vi "serial.vi"() -> ()   [LabVIEW 2017]
uses:
  <vilib>/Instr/_visa.llb/VISA Configure Serial Port (Instr).vi
panel:
  out "SUICHE":bool
  out "TEMPERATURA":dbl(slide) scale=0.0..100.0
  out "read buffer":string
  in  "PARAR":bool
  in  "PUERTO":refnum<visa-resource-name>="COM4"
  in  "Izquierda":bool
  in  "Derecha":bool
  in  "VELOCIDAD":dbl(knob) scale=0.0..100.0
  in  "LED2":bool
  in  "LED1":bool
  in  "stop":bool
  # "GIRO"
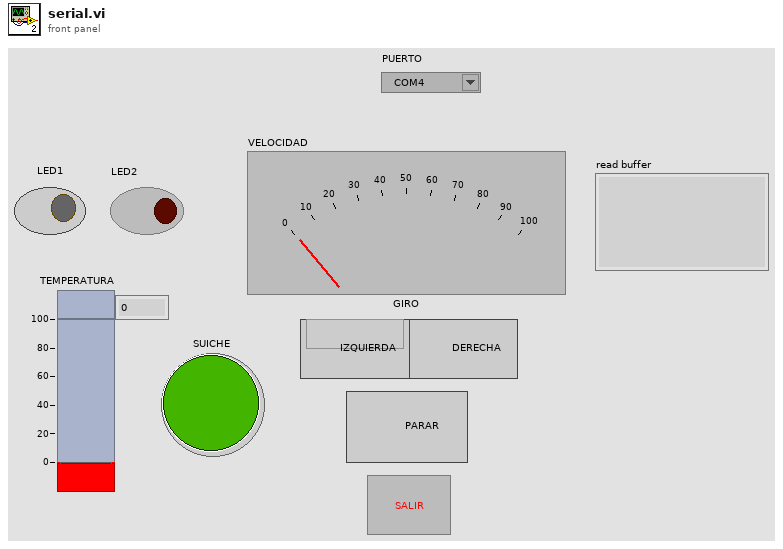
[diagram p1: front panel]
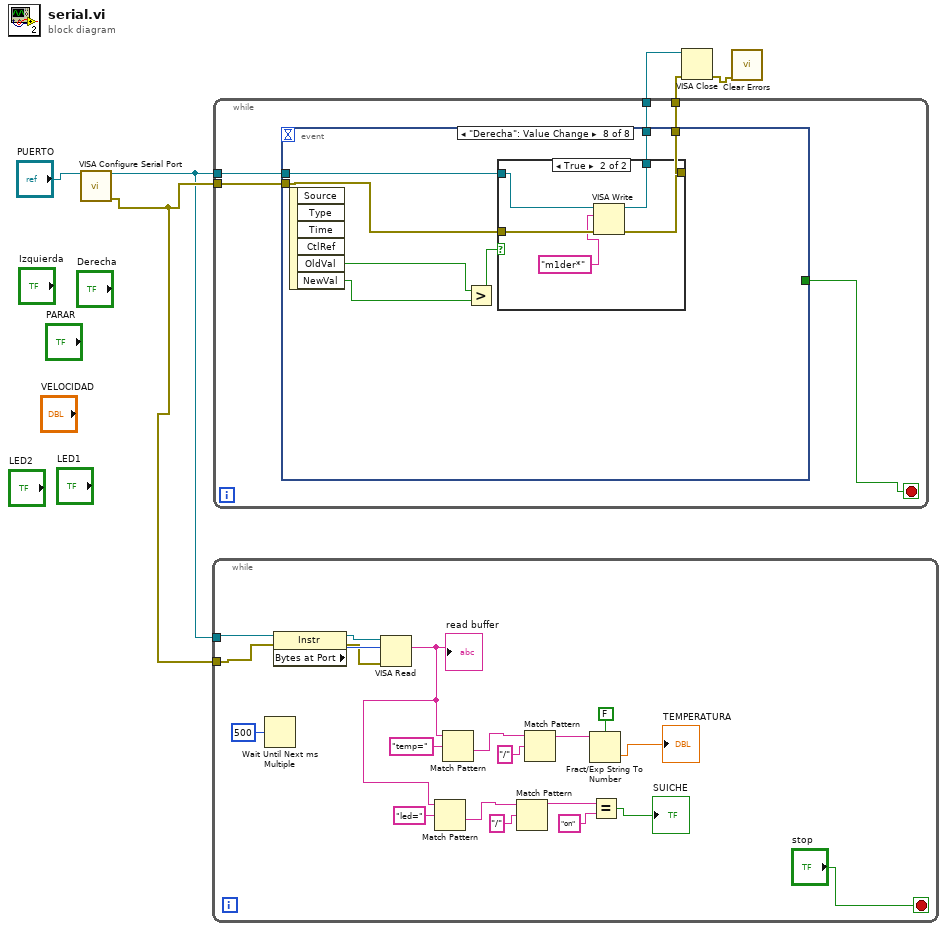
[diagram p0: block diagram]
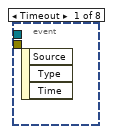
[diagram p2: hidden frame]
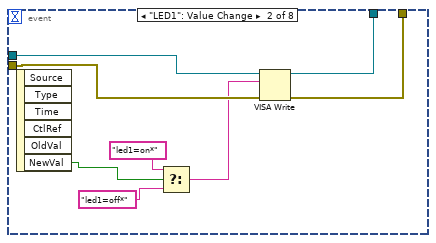
[diagram p3: hidden frame]
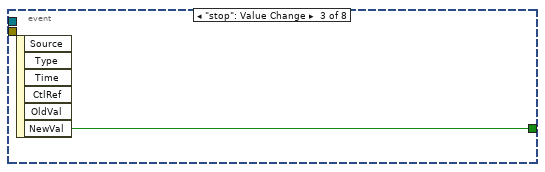
[diagram p4: hidden frame]
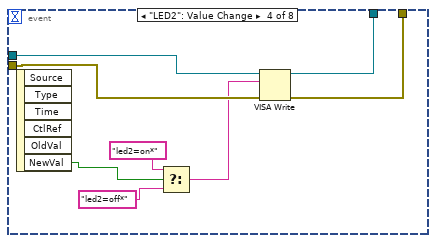
[diagram p5: hidden frame]
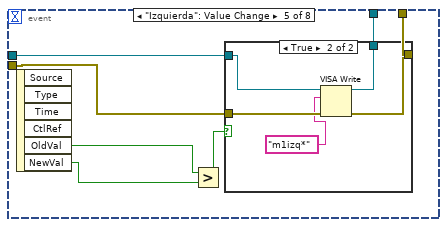
[diagram p6: hidden frame]
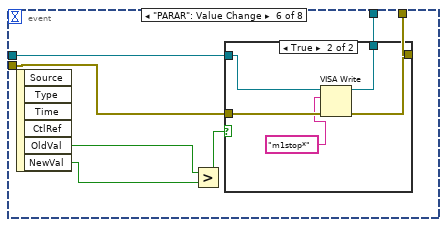
[diagram p8: hidden frame]
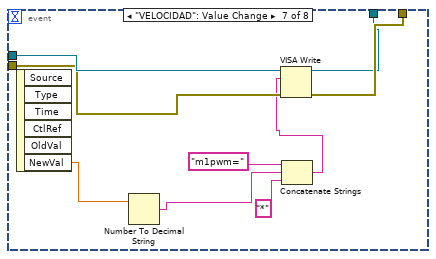
[diagram p10: hidden frame]
diagram:
  n1 = call-poly "VISA Configure Serial Port"("VISA resource name"="PUERTO") -> ("VISA resource name out"=w1:refnum<visa-resource-name>, "error out"=w2:errorcluster)  [unwired: 13 in]
  n2 = while {
    tunnel: w2 -> [w22]
    tunnel: w1 -> [w23]
    stop <- "stop" stop-if-true
    n3 = Wait Until Next ms Multiple(millisecond multiple=u32 500) -> ()  [unwired: 1 out]
    n4 = property class="Instr"(reference=w23, error in=w22) -> (reference out=w25:refnum<visa-resource-name>, error out=w24:errorcluster, "Bytes at Port"=w26:u32)
    n5 = VISA Read(VISA resource name=w25, byte count=w26, error in (no error)=w24) -> (read buffer=w9:string)  [unwired: 3 out]
    "read buffer" <- w9
    n6 = Match Pattern(string=w9, regular expression="led=") -> (after substring=w13:string)  [unwired: 1 in, 3 out]
    n7 = Match Pattern(string=w9, regular expression="temp=") -> (after substring=w19:string)  [unwired: 1 in, 3 out]
    n8 = Match Pattern(string=w13, regular expression="/") -> (before substring=w11:string)  [unwired: 1 in, 3 out]
    n9 = Match Pattern(string=w19, regular expression="/") -> (before substring=w17:string)  [unwired: 1 in, 3 out]
    n10 = Fract/Exp String To Number(use system decimal point (T)=FALSE, string=w17) -> (number=→"TEMPERATURA":dbl)  [unwired: 2 in, 1 out]
    n11 = Equal?(x=w11, y="on") -> (x = y?=→"SUICHE":bool)
  }
  n12 = while {
    tunnel: w1 -> [w31]
    tunnel: w2 -> [w30]
    tunnel: [w29] -> w5
    tunnel: [w28] -> w4
    stop <- w27 stop-if-true
    n13 = event shown="[7] \"Derecha\": Value Change" {
      selector: _ -> [_ _ _ _ _ _ _ _]
      dyn-events: _ -> [_ _ _ _ _ _ _ _]
      timeout: _ -> [_ _ _ _ _ _ _ _]
      tunnel: w31 -> [_ w39 _ w48 w55 w67 w81 w88]
      tunnel: w30 -> [_ w38 _ w47 w54 w66 w80 w87]
      tunnel: [_ w33 _ w42 w53 w65 w78 w86] -> w29
      tunnel: [_ w32 _ w41 w52 w64 w79 w85] -> w28
      tunnel: [_ _ w40 _ _ _ _ _] -> w27
      event Timeout {
        n14 = event-data() -> ()  [unwired: 1 in, 3 out]
      }
      event "LED1": Value Change {
        n15 = event-data() -> ("NewVal"=w37:bool)  [unwired: 1 in, 5 out]
        n16 = Select(t="led1=on*", s=w37, f="led1=off*") -> (s? t:f=w34:string)
        n17 = VISA Write(VISA resource name=w39, write buffer=w34, error in (no error)=w38) -> (VISA resource name out=w33:refnum<visa-resource-name>, error out=w32:errorcluster)  [unwired: 1 out]
      }
      event "stop": Value Change {
        n18 = event-data() -> ("NewVal"=w40:bool)  [unwired: 1 in, 5 out]
      }
      event "LED2": Value Change {
        n19 = event-data() -> ("NewVal"=w46:bool)  [unwired: 1 in, 5 out]
        n20 = Select(t="led2=on*", s=w46, f="led2=off*") -> (s? t:f=w43:string)
        n21 = VISA Write(VISA resource name=w48, write buffer=w43, error in (no error)=w47) -> (VISA resource name out=w42:refnum<visa-resource-name>, error out=w41:errorcluster)  [unwired: 1 out]
      }
      event "Izquierda": Value Change {
        n22 = event-data() -> ("OldVal"=w51:bool, "NewVal"=w50:bool)  [unwired: 1 in, 4 out]
        n23 = Greater?(x=w51, y=w50) -> (0:w49:bool)
        n24 = case shown="True" w49 {
          tunnel: w55 -> [_ w60]
          tunnel: w54 -> [_ w59]
          tunnel: [_ w58] -> w53
          tunnel: [_ w57] -> w52
          frame False {
          }
          frame True {
            n25 = VISA Write(VISA resource name=w60, write buffer="m1izq*", error in (no error)=w59) -> (VISA resource name out=w58:refnum<visa-resource-name>, error out=w57:errorcluster)  [unwired: 1 out]
          }
        }
      }
      event "PARAR": Value Change {
        n26 = event-data() -> ("OldVal"=w63:bool, "NewVal"=w62:bool)  [unwired: 1 in, 4 out]
        n27 = Greater?(x=w63, y=w62) -> (0:w61:bool)
        n28 = case shown="True" w61 {
          tunnel: w67 -> [_ w72]
          tunnel: w66 -> [_ w71]
          tunnel: [_ w70] -> w65
          tunnel: [_ w69] -> w64
          frame False {
          }
          frame True {
            n29 = VISA Write(VISA resource name=w72, write buffer="m1stop*", error in (no error)=w71) -> (VISA resource name out=w70:refnum<visa-resource-name>, error out=w69:errorcluster)  [unwired: 1 out]
          }
        }
      }
      event "VELOCIDAD": Value Change {
        n30 = event-data() -> ("NewVal"=w73:dbl)  [unwired: 1 in, 5 out]
        n31 = Number To Decimal String(number=w73) -> (decimal integer string=w76:string)  [unwired: 1 in]
        n32 = Concatenate Strings("m1pwm=" ("string"), w76, "*" ("string")) -> (w74:string)
        n33 = VISA Write(VISA resource name=w81, write buffer=w74, error in (no error)=w80) -> (VISA resource name out=w78:refnum<visa-resource-name>, error out=w79:errorcluster)  [unwired: 1 out]
      }
      event "Derecha": Value Change {
        n34 = event-data() -> ("OldVal"=w84:bool, "NewVal"=w83:bool)  [unwired: 1 in, 4 out]
        n35 = Greater?(x=w84, y=w83) -> (0:w82:bool)
        n36 = case shown="True" w82 {
          tunnel: w88 -> [_ w93]
          tunnel: w87 -> [_ w92]
          tunnel: [_ w91] -> w86
          tunnel: [_ w90] -> w85
          frame False {
          }
          frame True {
            n37 = VISA Write(VISA resource name=w93, write buffer="m1der*", error in (no error)=w92) -> (VISA resource name out=w91:refnum<visa-resource-name>, error out=w90:errorcluster)  [unwired: 1 out]
          }
        }
      }
    }
  }
  n38 = VISA Close(VISA resource name=w5, error in (no error)=w4) -> (error out=w3:errorcluster)
  n39 = call <vilib>:"Clear Errors.vi"("error in (no error)"=w3) -> ()  [unwired: 5 in, 2 out]
